vi "FuncVI2-Exec.vi"(4 "Caller CSE RefNum":T1, 5 "InstanceRef":T3, 9 "arg list":T2[](array[typedef]) {"num" format="%.2f"}) -> (0 "error out":bool, 3 "result":T2 {"num" format="%.2f"})   [LabVIEW 2021]
doc: "::: CalcExpress Toolkit :::\nCopyright (c) 2000-2026 Konstantin Shifershteyn. All rights reserved."
uses:
  cetypes.llb/CalcExpress Function Argument Info.ctl
  cetypes.llb/CalcExpress Instance RefNum.ctl
  cse.llb/CSE Instance RefNum.ctl
panel:
  in  "max arg num":i32=1
  in  "min arg num":i32=1
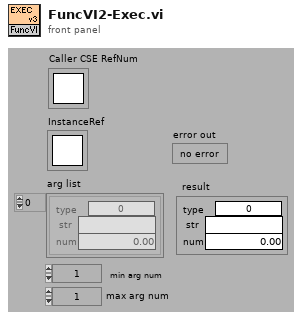
[diagram p1: front panel]
types:
  T1 = typedef "CSE Instance RefNum.ctl" = refnum<k1>
  T2 = typedef "CalcExpress Function Argument Info.ctl" = cluster{"type":u32, "str":string, "num":dbl}
  T3 = typedef "CalcExpress Instance RefNum.ctl" = refnum<k1>
  T4 = enum32{"String", "DBL Number", "identifier", "1D Array of DBL", "2D Array of DBL", "CDB Number", "1D Array of CDB", "2D Array of CDB", "1D Array of String", "2D Array of String", "Unknown data type"}
  T5 = typedef "CSE Callback VI RefNum.ctl" = refnum<vi>
  T6 = typedef "VarMan Variable Context Handle.ctl" = i32
  T7 = cluster{"type: use this constant to specify a predefined type code":enum32{"String", "DBL Number", "identifier", "1D Array of DBL", "2D Array of DBL", "CDB Number", "1D Array of CDB", "2D Array of CDB", "1D Array of String", "2D Array of String", "Unknown data type"}, string, "return value":dbl}
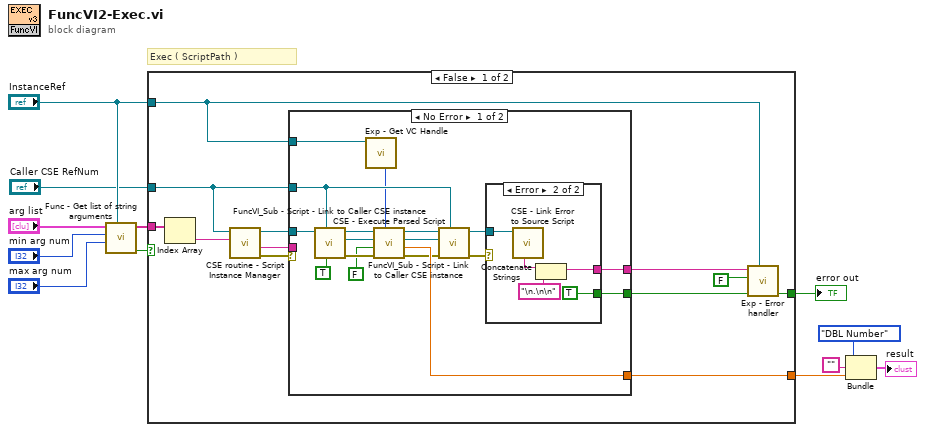
[diagram p0: block diagram]
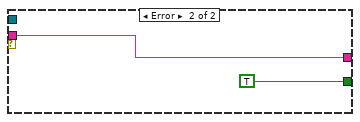
[diagram p3: hidden frame]
diagram:
  # "Exec ( ScriptPath )"
  n1 = call "Func - Get list of string arguments.vi"("InstanceRef"="InstanceRef", "max arg num"="max arg num", "min arg num"="min arg num", "arg list"="arg list") -> ("error out"=w7:bool, "val list"=w8:string[])  [unwired: 4 in]
  n2 = case shown="False" w7 {
    selector: w7 -> [_ w49]
    tunnel: "InstanceRef" -> [w19 _]
    tunnel: w8 -> [w18 _]
    tunnel: [w23 w49] -> w6
    tunnel: [w24 _] -> w2
    tunnel: "Caller CSE RefNum" -> [w16 _]
    frame False {
      n3 = Index Array(array=w18) -> (element=w17:string)  [unwired: 1 in]
      n4 = call "CSE routine - Script Instance Manager.vi"("Script Name"=w17, "Caller CSE RefNum"=w16) -> ("error out"=w15:errorcluster, "Error message"=w14:string, "new CSE RefNum"=w13:T1)  [unwired: 7 in]
      n5 = case shown="No Error" w15 {
        tunnel: [w41 _] -> w24
        tunnel: [w39 TRUE] -> w22
        tunnel: [w40 w48] -> w21
        tunnel: w16 -> [w30 _]
        tunnel: w19 -> [w27 _]
        tunnel: w14 -> [_ w48]
        tunnel: w13 -> [w26 _]
        frame No Error {
          n6 = call "FuncVI_Sub - Script - Link to Caller CSE instance.vi"("Link(T)/Delink(F)"=TRUE, "Caller CSE RefNum"=w30, "CSE RefNum"=w26) -> ("error out"=w33:errorcluster, "Callback VI RefNum out"=w34:T5, "dup CSE RefNum"=w35:T1)  [unwired: 6 in]
          n7 = call "Exp - Get VC Handle.vi"("InstanceRef"=w27) -> ("VC Handle"=w28:T6)  [unwired: 5 in, 3 out]
          n8 = call "CSE - Execute Parsed Script.vi"("VC Handle"=w28, "error in"=w33, "Close FuncVI Refs (T)"=FALSE, "Callback VI RefNum"=w34, "CSE RefNum"=w35) -> ("error out"=w31:errorcluster, "return value"=w41:dbl, "dup Callback VI RefNum"=w36:T5, "dup CSE RefNum"=w38:T1)  [unwired: 2 in, 1 out]
          n9 = call "FuncVI_Sub - Script - Link to Caller CSE instance.vi"("Caller CSE RefNum"=w30, "error in"=w31, "Callback VI RefNum"=w36, "CSE RefNum"=w38) -> ("error out"=w29:errorcluster, "dup CSE RefNum"=w37:T1)  [unwired: 5 in, 1 out]
          n10 = case shown="Error" w29 {
            tunnel: w37 -> [_ w46]
            tunnel: [_ TRUE] -> w39
            tunnel: [_ w42] -> w40
            frame No Error {
            }
            frame Error {
              n11 = call "CSE - Link Error to Source Script.vi"("CSE RefNum"=w46) -> ("Error Message"=w44:string)  [unwired: 4 in, 6 out]
              n12 = Concatenate Strings(w44, "\n.\n\n" ("string")) -> (w42:string)
            }
          }
        }
        frame Error {
        }
      }
      n13 = call "Exp - Error handler.vi"("InstanceRef"=w19, "error in"=w22, "add FuncName (T)"=FALSE, "error message in"=w21) -> ("error out"=w23:bool)  [unwired: 5 in, 2 out]
    }
    frame True {
    }
  }
  "error out" <- w6
  n14 = Bundle("type: use this constant to specify a predefined type code"=T4."DBL Number", "", "return value"=w2) -> (→"result":T7)  [unwired: 1 in]
